vi "CANsub_TLS_Connect.vi"(8 "error in (no error)":errorcluster, 9 "cert path":path=path "/home/lvuser/cansub_root_cert.crt", 10 "port":u16=443, 11 "host":string) -> (0 "error out":errorcluster, 2 "nodelay":i32, 3 "TLS connection":refnum<k5>)   [LabVIEW 2021, in "CANsub_Common.lvlib"]
doc: "Opens a TLS connection to the CANsub. Sets TCP_NODELAY on the socket before Start TLS and reads it back (nodelay must be 1, else error 5003). Trusts only the certificate in cert path. On an error before Start TLS, closes the TCP connection. The caller closes TLS connection with C7 CANsub_WS_Close. \n\nSets TCP keepalive (X5) before Start TLS.\n\nOn Windows the VI does not set TCP_NODELAY or keepalive; nodelay is 0."
uses:
  CANsub_Common.lvlib
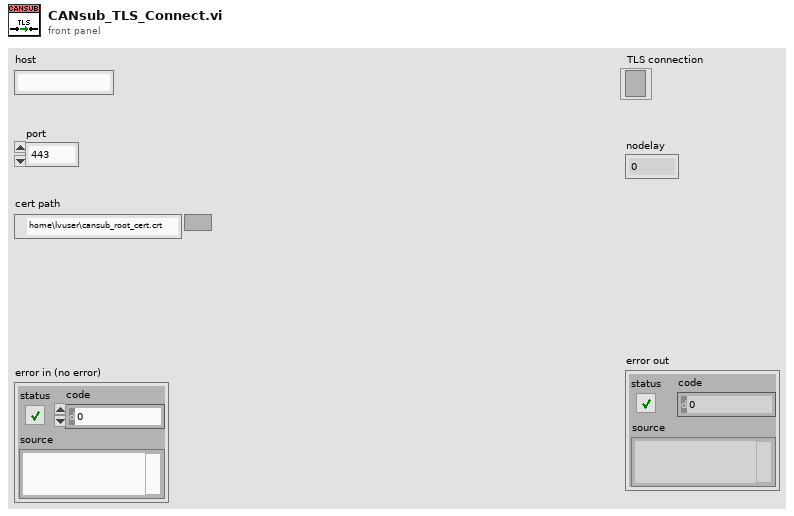
[diagram p1: front panel]
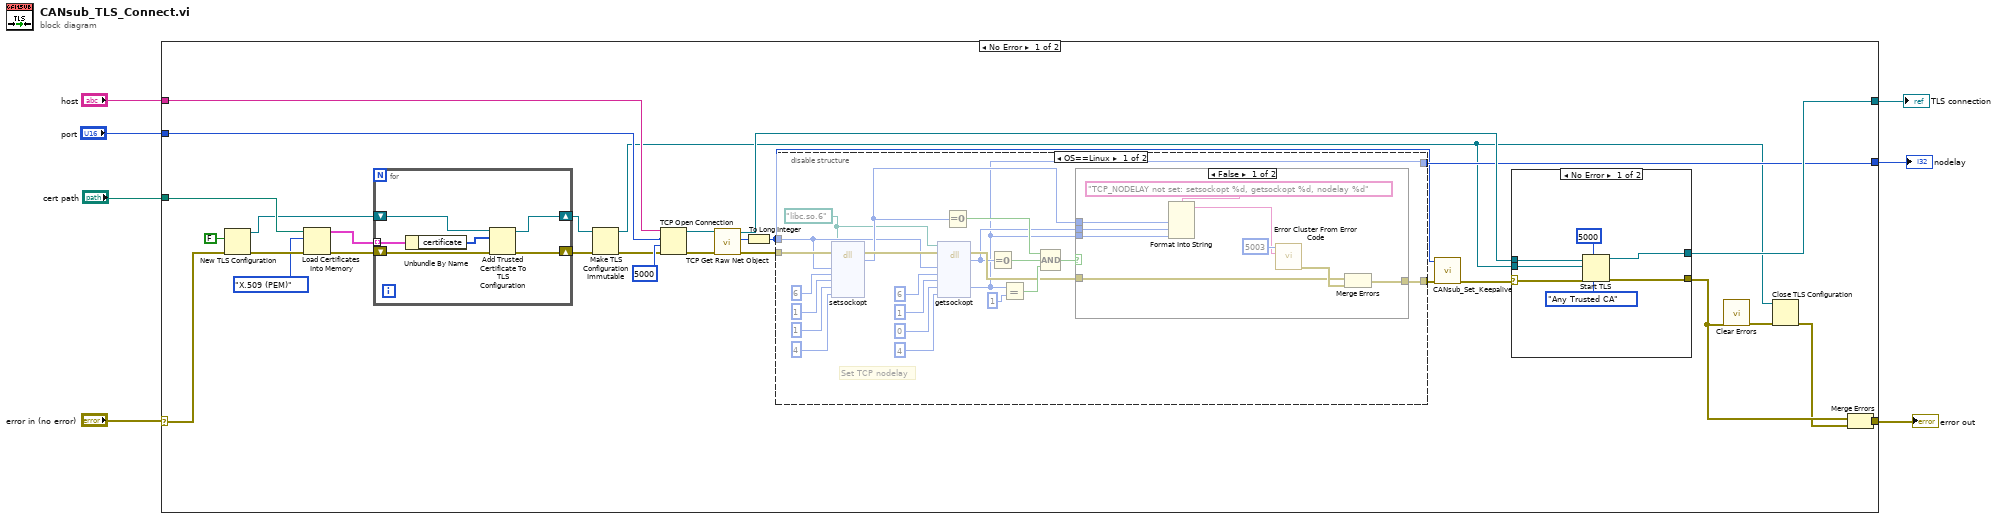
[diagram p0: block diagram]
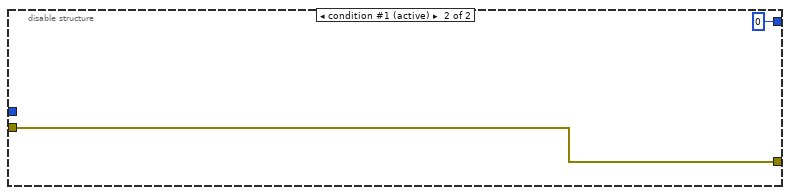
[diagram p3: hidden frame]
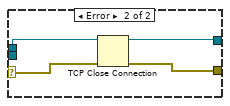
[diagram p4: hidden frame]
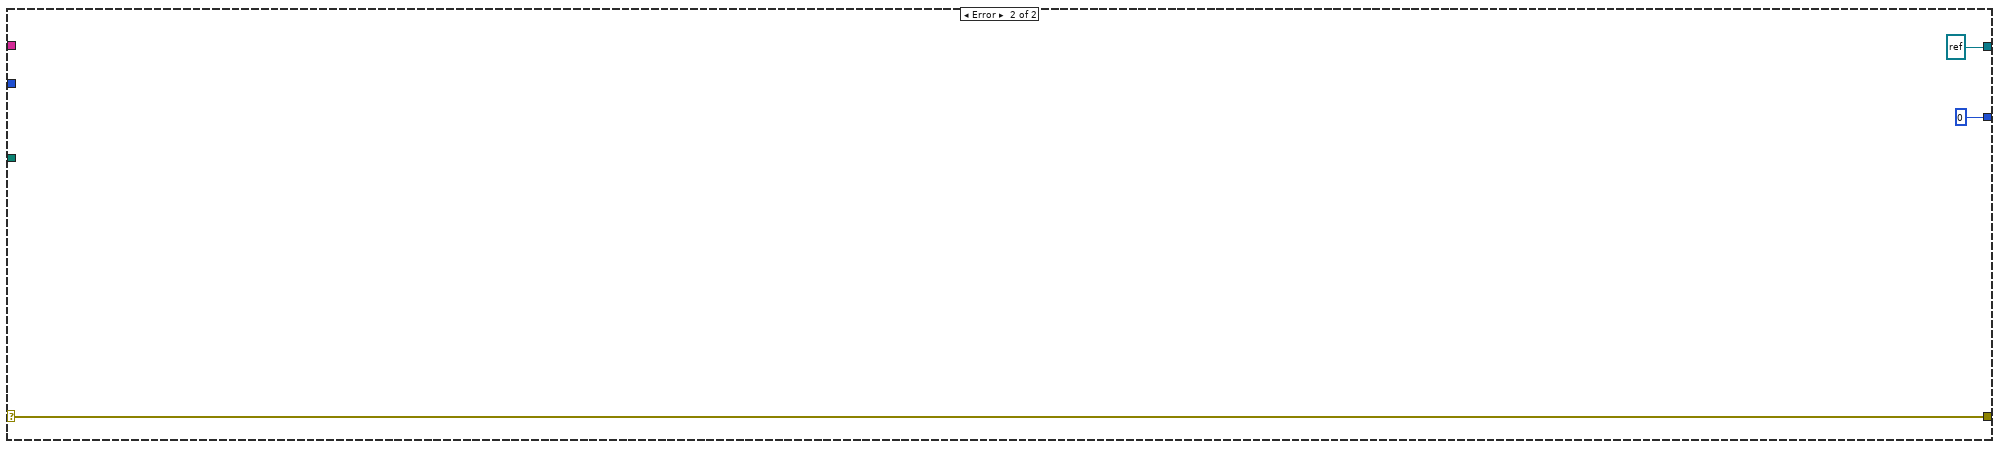
[diagram p5: hidden frame]
diagram:
  n1 = case shown="No Error" "error in (no error)" {
    selector: "error in (no error)" -> [w36 w90]
    tunnel: [w18 w90] -> w6
    tunnel: "cert path" -> [w34 _]
    tunnel: "host" -> [w28 _]
    tunnel: "port" -> [w27 _]
    tunnel: [w19 refnum<k5> refnum ("connection ID out")] -> w1
    tunnel: [w15 0 ("optval")] -> w2
    frame No Error {
      n2 = New TLS Configuration(8:w36, 10:FALSE ("load OS trusted CAs?")) -> (0:w35:errorcluster, 3:w31:refnum<k36>)
      n3 = Load Certificates Into Memory(8:w35, 10:enum32{"X.509 (PEM)"}."X.509 (PEM)" ("format"), 11:w34) -> (0:w30:errorcluster, 3:w32:cluster{"certificate":u8[]}[])
      n4 = for {
        tunnel: w32 -> [w83] mode=indexing
        shift-right: [w86] -> w11
        shift-left: w31 -> [w87]
        shift-right: [w85] -> w29
        shift-left: w30 -> [w84]
        n5 = Unbundle By Name(w83) -> ("certificate"=w82:u8[])
        n6 = Add Trusted Certificate To TLS Configuration(8:w84, 10:w82, 11:w87) -> (0:w85:errorcluster, 3:w86:refnum<k36>)
      }
      n7 = Make TLS Configuration Immutable(8:w29, 11:w11) -> (0:w25:errorcluster, 3:w13:refnum<k36>)
      n8 = TCP Open Connection(address=w28, remote port or service name=w27, timeout ms (60000)=5000, error in (no error)=w25) -> (connection ID=w23:refnum<k5>, error out=w24:errorcluster)  [unwired: 1 in]
      n9 = call <vilib>:"TCP Get Raw Net Object.vi"("error in (no error)"=w24, "connection ID"=w23) -> ("error out"=w21:errorcluster, "raw net object"=w22:u64, "connection ID out"=w20:refnum<k5>)  [unwired: 7 in]
      n10 = To Long Integer(number=w22) -> (32bit integer=w8:i32)
      n11 = disable-structure shown="OS==Linux" {
        disable-tunnel: w21 -> [w49 w70]
        disable-tunnel: [w40 0 ("optval")] -> w15
        disable-tunnel: [w39 w70] -> w10
        disable-tunnel: w8 -> [w38 _]
        frame condition #0 {
          w37 = path "libc.so.6" ("path in")
          # "Set TCP nodelay"
          n12 = dll-call lib="libc.so.6" fn="setsockopt"(path in=w37, error in=w49, "sockfd"=w38, "level"=6, "optname"=1, "optval"=1, "optlen"=u32 4) -> (error out=w58:errorcluster, "ret"=w42:i32)  [unwired: 6 in, 1 out]
          n13 = dll-call lib="libc.so.6" fn="getsockopt"(path in=w37, error in=w58, "sockfd"=w38, "level"=6, "optname"=1, "optval"=0, "optlen"=u32 4) -> (error out=w43:errorcluster, "ret"=w41:i32, "optval"=w40:i32)  [unwired: 5 in, 1 out]
          n14 = Equal To 0?(x=w42) -> (x = 0?=w45:bool)
          n15 = Equal To 0?(x=w41) -> (x = 0?=w46:bool)
          n16 = Equal?(x=w40, y=1) -> (x = y?=w47:bool)
          n17 = Compound Arithmetic op=AND(w45, w46, w47) -> (w44:bool)
          n18 = case shown="False" w44 {
            tunnel: w43 -> [w60 w68]
            tunnel: [w66 w68] -> w39
            tunnel: w42 -> [w64 _]
            tunnel: w41 -> [w63 _]
            tunnel: w40 -> [w62 _]
            frame False {
              n19 = Format Into String(format string="TCP_NODELAY not set: setsockopt %d, getsockopt %d, nodelay %d", w64, w63, w62) -> (resulting string=w59:string)  [unwired: 2 in, 1 out]
              n20 = call <vilib>:"Error Cluster From Error Code.vi"("error message (\"\")"=w59, "error code (0)"=5003) -> ("error out"=w67:errorcluster)  [unwired: 7 in]
              n21 = Merge Errors(w60, w67) -> (w66:errorcluster)
            }
            frame True {
            }
          }
        }
        frame condition #1 (active) {
        }
      }
      n22 = call "CANsub_Set_Keepalive.vi"("error in (no error)"=w10, "fd"=w8) -> ("error out"=w9:errorcluster)  [unwired: 8 in, 1 out]
      n23 = case shown="No Error" w9 {
        selector: w9 -> [w77 w80]
        tunnel: w20 -> [w75 w81]
        tunnel: [w71 w79] -> w19
        tunnel: [w76 w78] -> w17
        tunnel: w13 -> [w74 _]
        frame No Error {
          n24 = Start TLS(6:enum32{"Any Trusted CA", "None"}."Any Trusted CA" ("server certificate validation"), 7:5000 ("timeout ms"), 8:w77, 10:w74, 11:w75) -> (0:w76:errorcluster, 3:w71:refnum<k5>)  [unwired: 1 in, 1 out]
        }
        frame Error {
          n25 = TCP Close Connection(connection ID=w81, error in (no error)=w80) -> (connection ID out=w79:refnum<k5>, error out=w78:errorcluster)  [unwired: 1 in]
        }
      }
      n26 = call <vilib>:"Clear Errors.vi"("error in (no error)"=w17) -> ("error out"=w12:errorcluster)  [unwired: 5 in, 1 out]
      n27 = Close TLS Configuration(8:w12, 11:w13) -> (0:w16:errorcluster)
      n28 = Merge Errors(w17, w16) -> (w18:errorcluster)
    }
    frame Error {
    }
  }
  "error out" <- w6
  "TLS connection" <- w1
  "nodelay" <- w2
